vi "Output Parameter Type Constant Label--constant.vi"() -> (3 "Output Parameter Type Constant Label":string)   [LabVIEW 2026]
doc: "This constant defines the label of the cluster constant that defines the output for the python node."
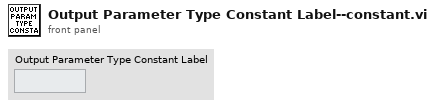
[diagram p1: front panel]
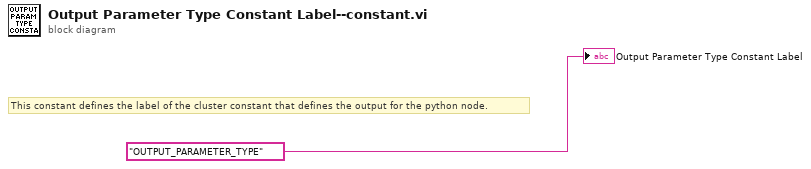
[diagram p0: block diagram]
diagram:
  # "This constant defines the label of the cluster constant that defines the output for the python node."
  "Output Parameter Type Constant Label" <- "OUTPUT_PARAMETER_TYPE" ("Function Name String Constant Label")
